vi "from string.vi"(8 "error in":errorcluster, 9 "data":string, 10 "version":string, 11 "PID Module configuration in":refnum<class "PID Module configuration.lvclass">) -> (0 "error out":errorcluster, 3 "PID Module configuration out":refnum<class "PID Module configuration.lvclass">)   [LabVIEW 2015, in "PID Module configuration.lvclass"]
doc: "Provides an interface for loading a module configuration from a file or other serialized data source. It is recommended that all children of this class store data in two sets--data required for its own initialization, and any data required for parent initialization--and that each implementation uses the <b>Call Parent Method</b> primitive to de-serialize parent information. As a result, it is expected that every module configuration class calls <b>component configuration.lvclass:From String.vi</b>."
uses:
  PID Module configuration.lvclass
  <vilib>/NI/Tag Bus Module Framework/module configuration/TBM module configuration.lvclass
  <vilib>/NI/Configuration Framework/serializable configuration/NISE_CEF_serializable configuration.lvclass
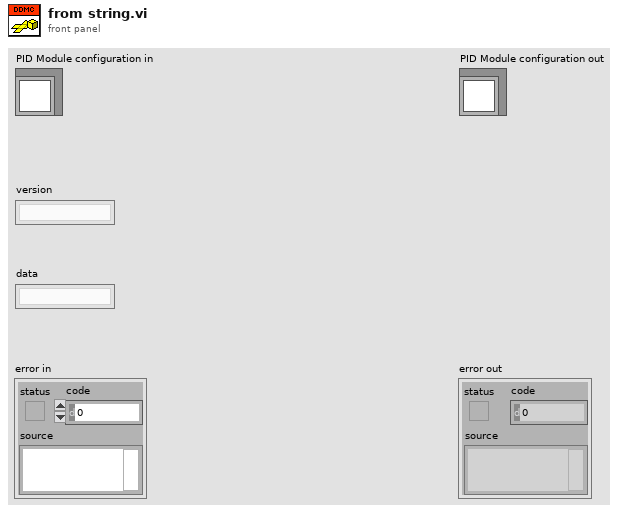
[diagram p1: front panel]
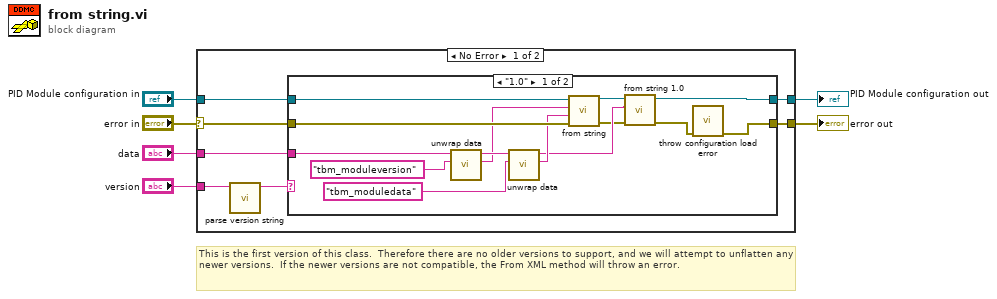
[diagram p0: block diagram]
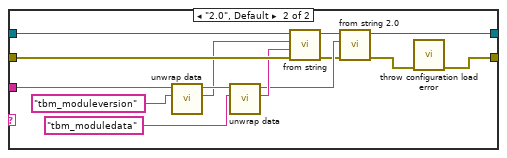
[diagram p2: hidden frame]
diagram:
  # "This is the first version of this class.  Therefore there are no older versions to support, and we will attempt to unflatten any newer versions.  If the newer versions are not compatible, the From XML method will throw an error."
  n1 = case shown="No Error" "error in" {
    selector: "error in" -> [w7 w43]
    tunnel: "data" -> [w13 _]
    tunnel: "PID Module configuration in" -> [w12 w42]
    tunnel: [w11 w42] -> w5
    tunnel: [w10 w43] -> w4
    tunnel: "version" -> [w9 _]
    frame No Error {
      n2 = call <vilib>:"parse version string.vi"("full version"=w9) -> ("major.minor version"=w8:string)  [unwired: 7 in, 3 out]
      n3 = case shown="\"1.0\"" w8 {
        tunnel: w13 -> [w24 w38]
        tunnel: w7 -> [w23 w37]
        tunnel: w12 -> [w27 w41]
        tunnel: [w16 w30] -> w11
        tunnel: [w26 w40] -> w10
        frame "1.0" {
          n4 = call <vilib>:"unwrap data.vi"("identifier"="tbm_moduleversion" ("additional identifier"), "data to unwrap"=w24) -> ("unwrapped data"=w19:string, "remaining string"=w25:string)  [unwired: 8 in]
          n5 = call <vilib>:"unwrap data.vi"("identifier"="tbm_moduledata" ("additional identifier"), "data to unwrap"=w25) -> ("unwrapped data"=w21:string, "remaining string"=w18:string)  [unwired: 8 in]
          n6 = call-parent "from string.vi"("error in"=w23, "data"=w21, "version"=w19, "module configuration in"=w27) -> ("error out"=w14:errorcluster, "module configuration out"=w17:refnum<class "PID Module configuration.lvclass">)  [unwired: 6 in]
          n7 = call "from string 1.0.vi"("error in (no error)"=w14, "data"=w18, "PID Module  configuration in"=w17) -> ("error out"=w15:errorcluster, "PID Module  configuration out"=w16:refnum<class "PID Module configuration.lvclass">)  [unwired: 7 in]
          n8 = call <vilib>:"throw configuration load error.vi"("error in"=w15) -> ("error out"=w26:errorcluster)  [unwired: 10 in]
        }
        frame "2.0", Default {
          n9 = call <vilib>:"unwrap data.vi"("identifier"="tbm_moduleversion" ("additional identifier"), "data to unwrap"=w38) -> ("unwrapped data"=w33:string, "remaining string"=w39:string)  [unwired: 8 in]
          n10 = call <vilib>:"unwrap data.vi"("identifier"="tbm_moduledata" ("additional identifier"), "data to unwrap"=w39) -> ("unwrapped data"=w35:string, "remaining string"=w32:string)  [unwired: 8 in]
          n11 = call-parent "from string.vi"("error in"=w37, "data"=w35, "version"=w33, "module configuration in"=w41) -> ("error out"=w29:errorcluster, "module configuration out"=w31:refnum<class "PID Module configuration.lvclass">)  [unwired: 6 in]
          n12 = call "from string 2.0.vi"("error in (no error)"=w29, "data"=w32, "PID Module configuration in"=w31) -> ("error out"=w28:errorcluster, "PID Module configuration out"=w30:refnum<class "PID Module configuration.lvclass">)  [unwired: 7 in]
          n13 = call <vilib>:"throw configuration load error.vi"("error in"=w28) -> ("error out"=w40:errorcluster)  [unwired: 10 in]
        }
      }
    }
    frame Error {
    }
  }
  "error out" <- w4
  "PID Module configuration out" <- w5
